vi "Test_Rules.vi"(11 "Rows":i32[](array[numeric])) -> ()   [LabVIEW 2026]
doc: "Rule_Check_Win / Rule_Check_Forbidden 테스트. Rows/Cols/Stones(1=흑,2=백)로 보드를 만들고 Move를 놓았을 때의 승리와 금수를 출력한다."
panel:
  out "error out":errorcluster
  out "Reason":T1(ring)
  out "Forbidden?":bool
  out "Run Length":i32
  out "Win Line":T2(array[cluster])
  out "Win?":bool
  in  "Renju":bool=TRUE
  in  "Exact Five":bool
  in  "Move Stone":i32=1
  in  "Move Col":i32=7
  in  "Move Row":i32=7
  in  "Stones":i32[](array[numeric])
  in  "Cols":i32[](array[numeric])
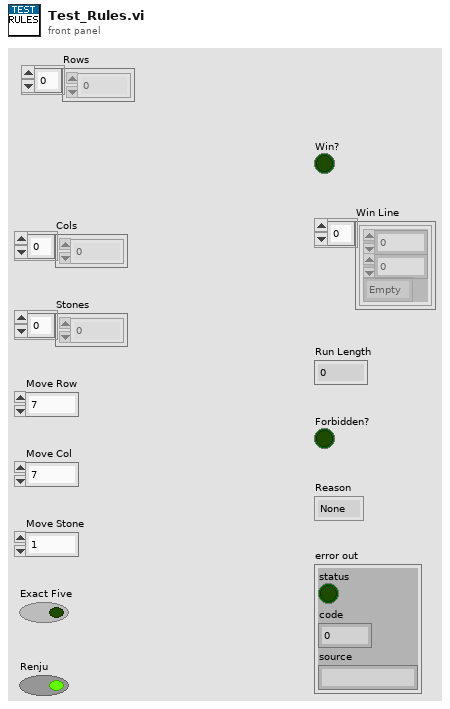
[diagram p1: front panel]
types:
  T1 = enum8{"None", "Double Three", "Double Four", "Overline"}
  T2 = cluster{"Row":i32, "Col":i32, "Stone":enum8{"Empty", "Black", "White"}}[]
  T3 = cluster{"Row":i32, "Col":i32, "Stone":enum8{"Empty", "Black", "White"}}
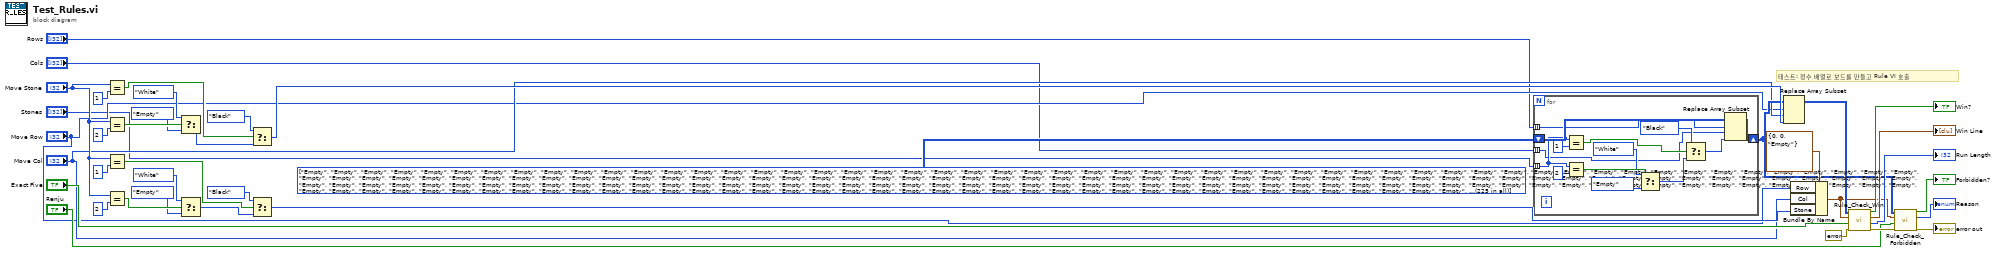
[diagram p0: block diagram]
diagram:
  w9 = enum8{"Empty", "Black", "White"}[][] [[enum."Empty", enum."Empty", enum."Empty", enum."Empty", enum."Empty", enum."Empty", enum."Empty", enum."Empty", enum."Empty", enum."Empty", enum."Empty", enum."Empty", enum."Empty", enum."Empty", enum."Empty"], [enum."Empty", enum."Empty", enum."Empty", enum."Empty", enum."Empty", enum."Empty", enum."Empty", enum."Empty", enum."Empty", enum."Empty", enum."Empty", enum."Empty", enum."Empty", enum."Empty", enum."Empty"], [enum."Empty", enum."Empty", enum."Empty", enum."Empty", enum."Empty", enum."Empty", enum."Empty", enum."Empty", enum."Empty", enum."Empty", enum."Empty", enum."Empty", enum."Empty", enum."Empty", enum."Empty"], [enum."Empty", enum."Empty", enum."Empty", enum."Empty", enum."Empty", enum."Empty", enum."Empty", enum."Empty", enum."Empty", enum."Empty", enum."Empty", enum."Empty", enum."Empty", enum."Empty", enum."Empty"], [enum."Empty", enum."Empty", enum."Empty", enum."Empty", enum."Empty", enum."Empty", enum."Empty", enum."Empty", enum."Empty", enum."Empty", enum."Empty", enum."Empty", enum."Empty", enum."Empty", enum."Empty"], [enum."Empty", enum."Empty", enum."Empty", enum."Empty", enum."Empty", enum."Empty", enum."Empty", enum."Empty", enum."Empty", enum."Empty", enum."Empty", enum."Empty", enum."Empty", enum."Empty", enum."Empty"], [enum."Empty", enum."Empty", enum."Empty", enum."Empty", enum."Empty", enum."Empty", enum."Empty", enum."Empty", enum."Empty", enum."Empty", enum."Empty", enum."Empty", enum."Empty", enum."Empty", enum."Empty"], [enum."Empty", enum."Empty", enum."Empty", enum."Empty", enum."Empty", enum."Empty", enum."Empty", enum."Empty", enum."Empty", enum."Empty", enum."Empty", enum."Empty", enum."Empty", enum."Empty", enum."Empty"], [enum."Empty", enum."Empty", enum."Empty", enum."Empty", enum."Empty", enum."Empty", enum."Empty", enum."Empty", enum."Empty", enum."Empty", enum."Empty", enum."Empty", enum."Empty", enum."Empty", enum."Empty"], [enum."Empty", enum."Empty", enum."Empty", enum."Empty", enum."Empty", enum."Empty", enum."Empty", enum."Empty", enum."Empty", enum."Empty", enum."Empty", enum."Empty", enum."Empty", enum."Empty", enum."Empty"], [enum."Empty", enum."Empty", enum."Empty", enum."Empty", enum."Empty", enum."Empty", enum."Empty", enum."Empty", enum."Empty", enum."Empty", enum."Empty", enum."Empty", enum."Empty", enum."Empty", enum."Empty"], [enum."Empty", enum."Empty", enum."Empty", enum."Empty", enum."Empty", enum."Empty", enum."Empty", enum."Empty", enum."Empty", enum."Empty", enum."Empty", enum."Empty", enum."Empty", enum."Empty", enum."Empty"], [enum."Empty", enum."Empty", enum."Empty", enum."Empty", enum."Empty", enum."Empty", enum."Empty", enum."Empty", enum."Empty", enum."Empty", enum."Empty", enum."Empty", enum."Empty", enum."Empty", enum."Empty"], [enum."Empty", enum."Empty", enum."Empty", enum."Empty", enum."Empty", enum."Empty", enum."Empty", enum."Empty", enum."Empty", enum."Empty", enum."Empty", enum."Empty", enum."Empty", enum."Empty", enum."Empty"], [enum."Empty", enum."Empty", enum."Empty", enum."Empty", enum."Empty", enum."Empty", enum."Empty", enum."Empty", enum."Empty", enum."Empty", enum."Empty", enum."Empty", enum."Empty", enum."Empty", enum."Empty"]] items=["Empty", "Black", "White"]
  # "테스트: 정수 배열로 보드를 만들고 Rule VI 호출"
  n1 = Equal?(x="Move Stone", y=1) -> (x = y?=w26:bool)
  n2 = Equal?(x="Move Stone", y=2) -> (x = y?=w28:bool)
  n3 = Equal?(x="Move Stone", y=1) -> (x = y?=w16:bool)
  n4 = Equal?(x="Move Stone", y=2) -> (x = y?=w18:bool)
  n5 = Select(t=enum8{"Empty", "Black", "White"}."White", s=w28, f=enum8{"Empty", "Black", "White"}."Empty") -> (s? t:f=w29:enum8{"Empty", "Black", "White"})
  n6 = Select(t=enum8{"Empty", "Black", "White"}."White", s=w18, f=enum8{"Empty", "Black", "White"}."Empty") -> (s? t:f=w19:enum8{"Empty", "Black", "White"})
  n7 = Select(t=enum8{"Empty", "Black", "White"}."Black", s=w26, f=w29) -> (s? t:f=w30:enum8{"Empty", "Black", "White"})
  n8 = Select(t=enum8{"Empty", "Black", "White"}."Black", s=w16, f=w19) -> (s? t:f=w20:enum8{"Empty", "Black", "White"})
  n9 = for {
    tunnel: "Rows" -> [w40] mode=indexing
    tunnel: "Cols" -> [w41] mode=indexing
    tunnel: "Stones" -> [w42] mode=indexing
    shift-right: [w52] -> w10
    shift-left: w9 -> [w53]
    n10 = Equal?(x=w42, y=1) -> (x = y?=w47:bool)
    n11 = Equal?(x=w42, y=2) -> (x = y?=w49:bool)
    n12 = Select(t=enum8{"Empty", "Black", "White"}."White", s=w49, f=enum8{"Empty", "Black", "White"}."Empty") -> (s? t:f=w50:enum8{"Empty", "Black", "White"})
    n13 = Select(t=enum8{"Empty", "Black", "White"}."Black", s=w47, f=w50) -> (s? t:f=w51:enum8{"Empty", "Black", "White"})
    n14 = Replace Array Subset(array=w53, new element=w51, index (row)=w40, index (col)=w41) -> (w52:enum8{"Empty", "Black", "White"}[][])
  }
  n15 = Replace Array Subset(array=w10, new element=w30, index (row)="Move Row", index (col)="Move Col") -> (w31:enum8{"Empty", "Black", "White"}[][])
  n16 = Bundle By Name(cluster=T3 {"Row"=0, "Col"=0, "Stone"=enum."Empty"}, "Row"="Move Row", "Col"="Move Col", "Stone"=w20) -> (w21:T3)
  n17 = call "Rule_Check_Win.vi"("error in"=errorcluster {"status"=FALSE, "code"=0, "source"=""}, "Exact Five"="Exact Five", "Last Move"=w21, "Grid"=w31) -> ("error out"=w36:errorcluster, "Run Length"=→"Run Length":i32, "Win Line"=→"Win Line":T2, "Win?"=→"Win?":bool)  [unwired: 4 in]
  n18 = call "Rule_Check_Forbidden.vi"("error in"=w36, "Renju"="Renju", "Move"=w21, "Grid"=w10) -> ("error out"=→"error out":errorcluster, "Reason"=→"Reason":T1, "Forbidden?"=→"Forbidden?":bool)  [unwired: 5 in]
